vi "Update Sort Column.vi"(6 "Reset?":bool, 8 "error in":errorcluster, 10 "Cell Position":T1, 11 "Peer Review in":refnum<class "Peer Review.lvclass">) -> (0 "error out":errorcluster, 3 "Peer Review out":refnum<class "Peer Review.lvclass">)   [LabVIEW 2020, in "Peer Review.lvclass"]
uses:
  Peer Review.lvclass
  <vilib>/Utility/miscctls.llb/LVRowAndColumnTypeDef.ctl
  Peer Review.lvclass/Peer Review.ctl
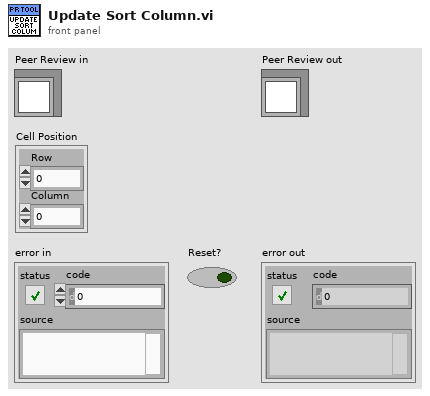
[diagram p1: front panel]
types:
  T1 = typedef "LVRowAndColumnTypeDef.ctl" = cluster{"Row":i32, "Column":i32}
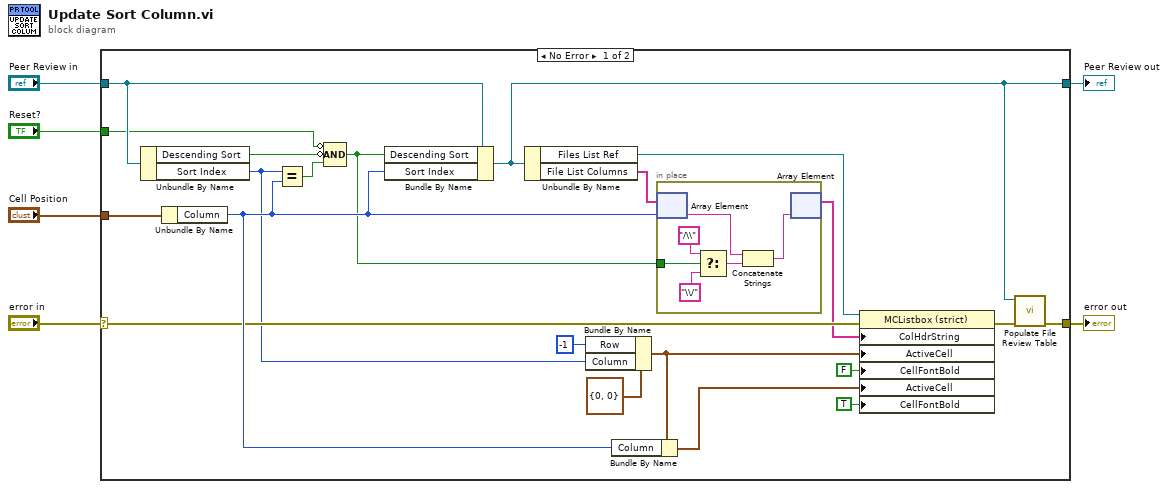
[diagram p0: block diagram]
diagram:
  n1 = case shown="No Error" "error in" {
    selector: "error in" -> [w22 w35]
    tunnel: [w27 w35] -> w5
    tunnel: "Cell Position" -> [w23 _]
    tunnel: "Peer Review in" -> [w25 w34]
    tunnel: [w24 w34] -> w2
    tunnel: "Reset?" -> [w21 _]
    frame No Error {
      n2 = Unbundle By Name(w25) -> ("Descending Sort"=w12:bool, "Sort Index"=w13:i32)
      n3 = Unbundle By Name(w23) -> ("Column"=w26:i32)
      n4 = Equal?(x=w13, y=w26) -> (x = y?=w15:bool)
      n5 = Compound Arithmetic op=AND(invert w21, invert w12, w15) -> (w7:bool)
      n6 = Bundle By Name(cluster=w25, "Descending Sort"=w7, "Sort Index"=w26) -> (w24:refnum<class "Peer Review.lvclass">)
      n7 = Unbundle By Name(w24) -> ("Files List Ref"=w11:refnum<vi>, "File List Columns"=w10:string[])
      n8 = Bundle By Name(cluster=T1 {"Row"=0, "Column"=0} ("Active Cell:Active Cell"), "Row"=-1, "Column"=w13) -> (w16:T1)
      n9 = Bundle By Name(cluster=w16, "Column"=w26) -> (w9:T1)
      n10 = in-place {
        in-place-border: w7 -> [w30]
        n11 = in-place-array #1(w10, w26) -> (w29:string)
        n12 = Select(t="/\\" ("y"), s=w30, f="\\/" ("y")) -> (s? t:f=w33:string)
        n13 = Concatenate Strings(w29, w33) -> (w28:string)
        n14 = in-place-array #1(w28) -> (w14:string[])  [unwired: 1 out]
      }
      n15 = property on="Property Node" class="MCListbox (strict)"(reference=w11, error in=w22, "ColHdrString"=w14, "ActiveCell"=w16, "CellFontBold"=FALSE ("Active Cell:Cell Font:Bold"), "ActiveCell"=w9, "CellFontBold"=TRUE ("Active Cell:Cell Font:Bold")) -> (error out=w8:errorcluster)  [unwired: 1 out]
      n16 = call "Populate File Review Table.vi"("error in"=w8, "Peer Review"=w24) -> ("error out"=w27:errorcluster)  [unwired: 9 in]
    }
    frame Error {
    }
  }
  "error out" <- w5
  "Peer Review out" <- w2
